vi "CE Client - Run CE Server at Local Machine.vi"(8 "error in":errorcluster, 11 "machine name":string) -> (0 "error out":errorcluster, 3 "dup machine name":string)   [LabVIEW 2021]
doc: "::: CalcExpress Toolkit :::\nCopyright (c) 2000-2026 Konstantin Shifershteyn. All rights reserved."
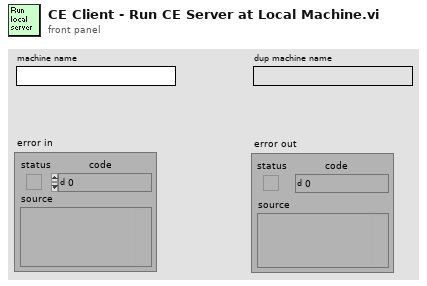
[diagram p1: front panel]
types:
  T1 = enum32{"Bad", "Idle", "Run top level", "Running"}
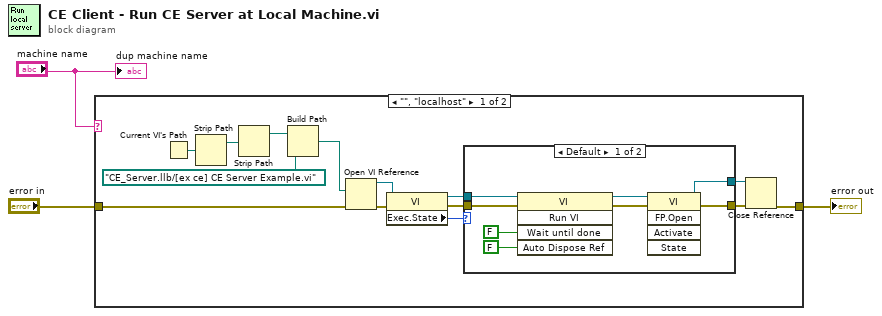
[diagram p0: block diagram]
diagram:
  n1 = case shown="\"\", \"localhost\"" "machine name" {
    tunnel: "error in" -> [w5 w28]
    tunnel: [w4 w28] -> w1
    frame "", "localhost" {
      n2 = Current VI's Path() -> (path=w6:path)
      n3 = Strip Path(path=w6) -> (stripped path=w7:path)  [unwired: 1 out]
      n4 = Strip Path(path=w7) -> (stripped path=w8:path)  [unwired: 1 out]
      n5 = Build Path(base path=w8, name or relative path=path "CE_Server.llb/[ex ce] CE Server Example.vi") -> (appended path=w10:path)
      n6 = Open VI Reference(vi path=w10, error in (no error)=w5) -> (vi reference=w12:refnum<vi>, error out=w11:errorcluster)  [unwired: 4 in]
      n7 = property class="VI"(reference=w12, error in=w11) -> (reference out=w14:refnum<vi>, error out=w17:errorcluster, "Exec.State"=w13:T1)
      n8 = case shown="Default" w13 {
        tunnel: w14 -> [w25 w26]
        tunnel: [w21 w27] -> w15
        tunnel: [w20 w26] -> w16
        tunnel: w17 -> [w19 w27]
        frame Default {
          n9 = invoke class="VI" method="Run VI"(reference=w25, error in=w19, "Wait until done"=FALSE ("Wait Until Done"), "Auto Dispose Ref"=FALSE ("Auto Dispose Reference")) -> (reference out=w22:refnum<vi>, error out=w18:errorcluster)  [unwired: 1 in, 3 out]
          n10 = invoke class="VI" method="FP.Open"(reference=w22, error in=w18) -> (reference out=w20:refnum<vi>, error out=w21:errorcluster)  [unwired: 3 in, 3 out]
        }
        frame "Run top level" {
        }
      }
      n11 = Close Reference(reference=w16, error in (no error)=w15) -> (error out=w4:errorcluster)
    }
    frame Default {
    }
  }
  "error out" <- w1
  "dup machine name" <- "machine name"
